vi "Set PWM.Balance.vi"(7 "PWM Clock Divider":i32=1024, 8 "error in (no error)":errorcluster, 9 "Duty Cycle (0-1)":dbl=0.5, 10 "PWM Freq (Hz)":dbl=50.0, 11 "RPi PWM Pin in":T1=enum."GPIO12_PWM0_Pin32") -> (0 "error out":errorcluster, 1 "Actual Duty-Cycle":dbl, 2 "Actual Period":dbl=100.0, 3 "RPi PWM Pin out":T1=enum."GPIO12_PWM0_Pin32", 5 "PWM Timing":cluster{"PWM Range":u32, "PWM Data":u32})   [LabVIEW 2020, in "wiringPi.lvlib"]
doc: "<b>_______________________________________________________________</b>\n** Author: Juan José Villacorta\n** LabVIEW wrapper for C library <b> wiringPi </b>,\n** https://github.com/WiringPi/WiringPi\n<b>_______________________________________________________________</b>\n\nSet the PWM frequency and duty-cycle"
uses:
  wiringPi.lvlib
  Type Defs/PWM Mode.ctl
  Type Defs/GPIO Pins.ctl
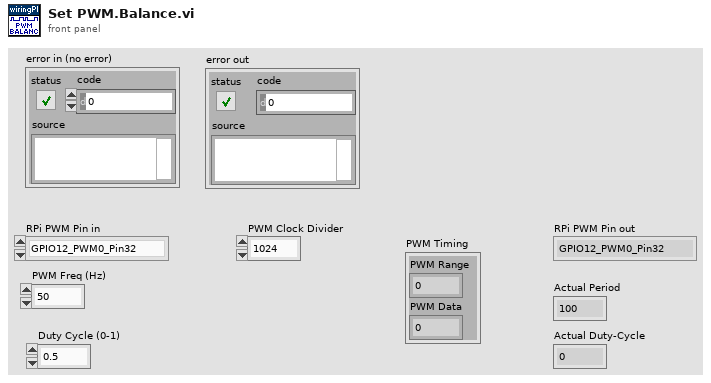
[diagram p1: front panel]
types:
  T1 = typedef "wiringPi.lvlib/GPIO Pins.ctl" = enum32{"GPIO0_I2C0_SDA_Pin27", "GPIO1_I2C0_SDA1_Pin28", "GPIO2_I2C1_SDA_Pin3", "GPIO3_I2C1_SCL_Pin5", "GPIO4_GPCLK0_Pin7", "GPIO5_GPCLK1_Pin29", "GPIO6_GPCLK2_Pin31", "GPIO7_SPI_CE1_N_Pin26", "GPIO8_SPI_CE0_N_Pin24", "GPIO9_SPI0_MISO_Pin21", "GPIO10_SPI0_MOSI_Pin19", "GPIO11_SPI0_CLK_Pin23", "GPIO12_PWM0_Pin32", "GPIO13_PWM1_Pin33", "GPIO14_TXD0_Pin8", "GPIO15_RXD0_Pin10", "GPIO16_Pin36", "GPIO17_Pin11", "GPIO18_PWM0_Pin12", "GPIO19_PWM1_Pin35", "GPIO20_GPCLK0_Pin38", "GPIO21_GPCLK1_Pin40", "GPIO22_Pin15", "GPIO23_Pin16", "GPIO24_Pin18", "GPIO25_Pin22", "GPIO26_Pin37", "GPIO27_Pin13"}
  T2 = typedef "wiringPi.lvlib/PWM Mode.ctl" = enum16{"Mark/Space", "Balanced"}
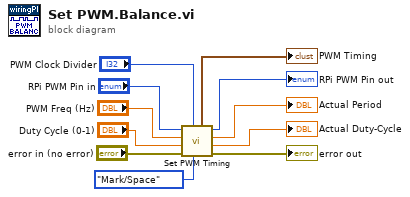
[diagram p0: block diagram]
diagram:
  n1 = call "Set PWM Timing.vi"("PWM Mode"=PWM_Mode."Mark/Space", "PWM Clock Divider"="PWM Clock Divider", "error in (no error)"="error in (no error)", "Duty Cycle"="Duty Cycle (0-1)", "PWM Freq"="PWM Freq (Hz)", "RPi PWM Pin in"="RPi PWM Pin in") -> ("error out"=→"error out":errorcluster, "Actual Duty-Cycle"=→"Actual Duty-Cycle":dbl, "Actual Period"=→"Actual Period":dbl, "RPi PWM Pin out"=→"RPi PWM Pin out":T1, "PWM Timing"=→"PWM Timing":cluster{"PWM Range":u32, "PWM Data":u32})  [unwired: 1 in]
